vi "set Meas Preset - 9020A.vi"(8 "error in (no error)":errorcluster, 10 "Measurement Preset":T1, 11 "Keysight 9020A in":refnum<class "Keysight 9020A.lvclass">) -> (0 "error out":errorcluster, 3 "Keysight 9020A out":refnum<class "Keysight 9020A.lvclass">)   [LabVIEW 2023, in "Spectrum Analyzer.lvlib" / "Keysight 9020A.lvclass"]
uses:
  Keysight 9020A.lvclass
  TYPE DEFINITION/Keysight 9020A/TYPE Measurement Preset.ctl
  Keysight 9020A.lvclass/Keysight 9020A.ctl
  Spectrum Analyzer.lvlib
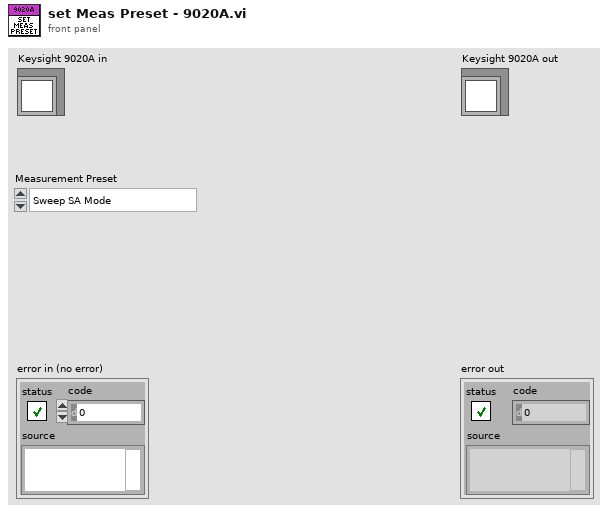
[diagram p1: front panel]
types:
  T1 = typedef "Spectrum Analyzer.lvlib/TYPE Measurement Preset.ctl" = enum16{"Sweep SA Mode", "Channel Power", "Occupied BW", "ACP", "Spurious Emission", "Spurious Emission Mask", "Burst Power (Transmit Power)"}
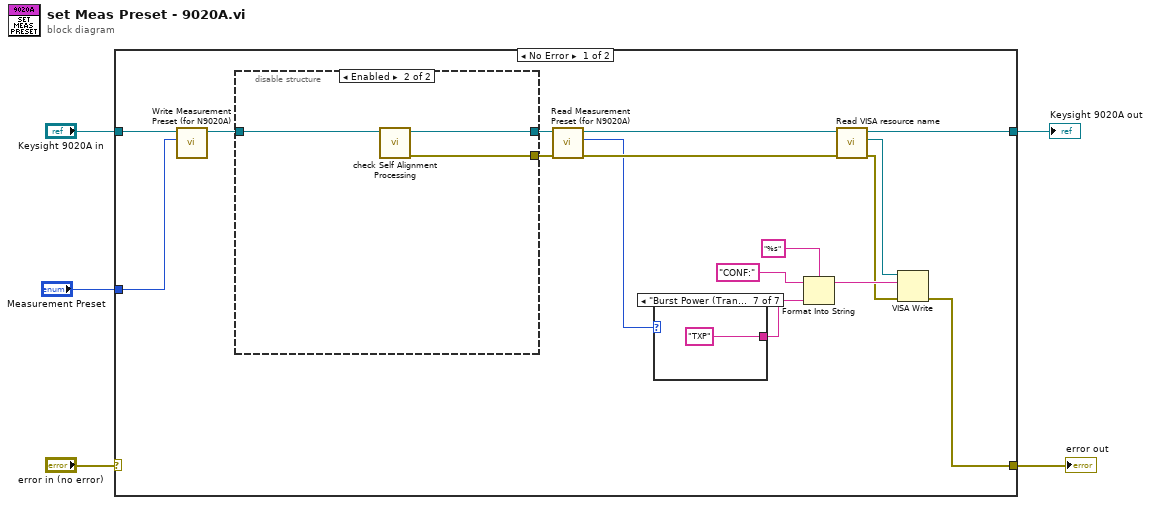
[diagram p0: block diagram]
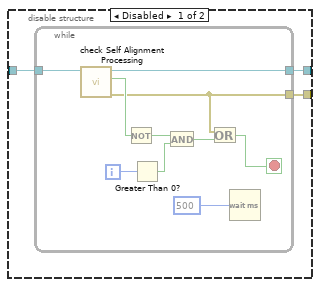
[diagram p2: hidden frame]
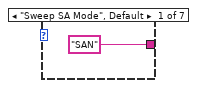
[diagram p3: hidden frame]
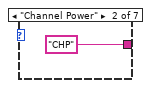
[diagram p4: hidden frame]
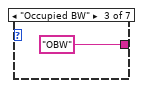
[diagram p5: hidden frame]
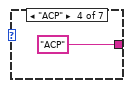
[diagram p6: hidden frame]
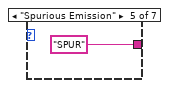
[diagram p7: hidden frame]
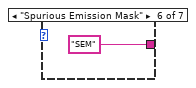
[diagram p8: hidden frame]
diagram:
  n1 = case shown="No Error" "error in (no error)" {
    selector: "error in (no error)" -> [_ w45]
    tunnel: "Keysight 9020A in" -> [w8 w46]
    tunnel: [w21 w46] -> w2
    tunnel: [w17 w45] -> w3
    tunnel: "Measurement Preset" -> [w7 _]
    frame No Error {
      n2 = call "Write Measurement Preset (for N9020A).vi"("Measurement Preset"=w7, "Keysight 9020A in"=w8) -> ("Keysight 9020A out"=w6:refnum<class "Keysight 9020A.lvclass">)  [unwired: 8 in, 1 out]
      n3 = disable-structure shown="Enabled" {
        disable-tunnel: [w24 w36] -> w13
        disable-tunnel: [w23 w35] -> w12
        disable-tunnel: w6 -> [w22 w37]
        frame Disabled {
          n4 = while {
            tunnel: w22 -> [w34]
            tunnel: [w28] -> w23
            tunnel: [w26] -> w24
            i -> [w31]
            stop <- w27 stop-if-true
            n5 = call "check Self Alignment Processing.vi"("Keysight 9020A in"=w34) -> ("error out"=w28:errorcluster, "On Alignment Processing"=w33:bool, "Keysight 9020A out"=w26:refnum<class "Keysight 9020A.lvclass">)  [unwired: 8 in]
            n6 = Not(x=w33) -> (.not. x?=w32:bool)
            n7 = Greater Than 0?(x=w31) -> (x > 0?=w30:bool)
            n8 = And(x=w32, y=w30) -> (x .and. y?=w29:bool)
            n9 = Or(x=w28, y=w29) -> (x .or. y?=w27:bool)
            n10 = Wait (ms)(milliseconds to wait=u32 500) -> ()  [unwired: 1 out]
          }
        }
        frame Enabled {
          n11 = call "check Self Alignment Processing.vi"("Keysight 9020A in"=w37) -> ("error out"=w35:errorcluster, "Keysight 9020A out"=w36:refnum<class "Keysight 9020A.lvclass">)  [unwired: 8 in, 1 out]
        }
      }
      n12 = call "Read Measurement Preset (for N9020A).vi"("error in (no error)"=w12, "Keysight 9020A in"=w13) -> ("error out"=w10:errorcluster, "Measurement Preset"=w9:T1, "Keysight 9020A out"=w11:refnum<class "Keysight 9020A.lvclass">)  [unwired: 7 in]
      n13 = case shown="\"Burst Power (Transmit Power)\"" w9 {
        tunnel: ["SAN" ("write buffer") "CHP" ("write buffer") "OBW" ("write buffer") "ACP" ("write buffer") "SPUR" ("write buffer") "SEM" ("write buffer") "TXP" ("write buffer")] -> w16
        frame "Sweep SA Mode", Default {
        }
        frame "Channel Power" {
        }
        frame "Occupied BW" {
        }
        frame "ACP" {
        }
        frame "Spurious Emission" {
        }
        frame "Spurious Emission Mask" {
        }
        frame "Burst Power (Transmit Power)" {
        }
      }
      n14 = Format Into String(format string="%s", initial string="CONF:", w16) -> (resulting string=w18:string)  [unwired: 1 in, 1 out]
      n15 = call "Read VISA resource name.vi"("error in (no error)"=w10, "Keysight 9020A in"=w11) -> ("error out"=w14:errorcluster, "VISA resource name"=w15:refnum<visa-resource-name>, "Keysight 9020A out"=w21:refnum<class "Keysight 9020A.lvclass">)  [unwired: 7 in]
      n16 = VISA Write(VISA resource name=w15, write buffer=w18, error in (no error)=w14) -> (error out=w17:errorcluster)  [unwired: 2 out]
    }
    frame Error {
    }
  }
  "error out" <- w3
  "Keysight 9020A out" <- w2
